vi "demo3.vi"() -> ()   [LabVIEW 2026]
uses:
  My Singleton Module.lvlib
panel:
  out "Gauge":dbl(knob) scale=0.0..10.0
  out "Status":string
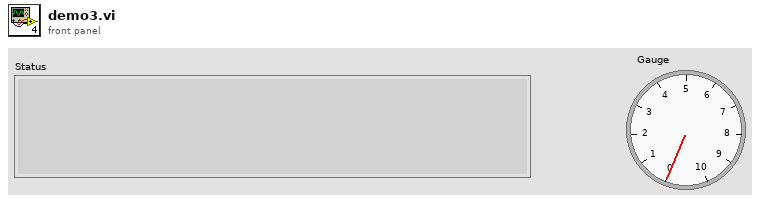
[diagram p1: front panel]
types:
  T1 = typedef "My Singleton Module.lvlib/Broadcast Events--cluster.ctl" = cluster{"Module Did Init":refnum<user-event>, "Status Updated":refnum<user-event>, "Error Reported":refnum<user-event>, "Did Something":refnum<user-event>, "Module Did Stop":refnum<user-event>, "Update Module Execution Status":refnum<user-event>, "Nuevo resultado de la Suma Actualizado":refnum<user-event>}
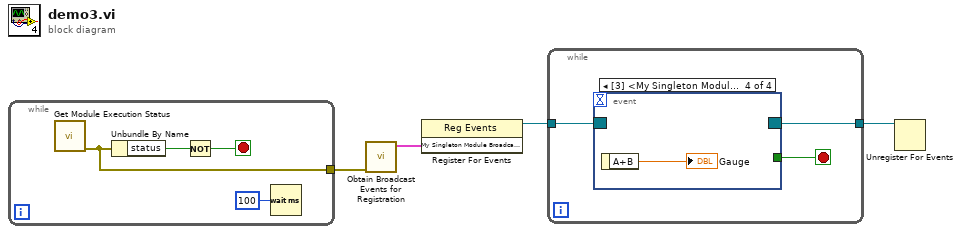
[diagram p0: block diagram]
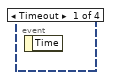
[diagram p2: hidden frame]
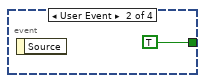
[diagram p3: hidden frame]
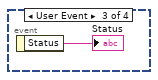
[diagram p4: hidden frame]
diagram:
  n1 = while {
    tunnel: [w5] -> w1
    stop <- w6 stop-if-true
    n2 = call "Get Module Execution Status.vi"() -> ("error out"=w5:errorcluster)  [unwired: 11 in]
    n3 = Unbundle By Name(w5) -> ("status"=w7:bool)
    n4 = Not(x=w7) -> (.not. x?=w6:bool)
    n5 = Wait (ms)(milliseconds to wait=u32 100) -> ()  [unwired: 1 out]
  }
  n6 = call "Obtain Broadcast Events for Registration.vi"("error in"=w1) -> ("My Singleton Module Broadcast Events"=w4:T1)  [unwired: 8 in, 2 out]
  n7 = register-events(w4) -> (reference out=w3:refnum<event-registration>)  [unwired: 2 in, 1 out]
  n8 = while {
    tunnel: w3 -> [w11]
    tunnel: [w9] -> w2
    stop <- w10 stop-if-true
    n9 = event shown="[3] <My Singleton Module Broadcast Events.Nuevo resultado de la Suma Actualizado>: User Event" {
      selector: w11 -> [_ _ _ _]
      dyn-events: [_ _ _ _] -> w9
      timeout: _ -> [_ _ _ _]
      tunnel: [_ TRUE _ _] -> w10
      event Timeout {
        n10 = event-data() -> ()  [unwired: 1 in, 1 out]
      }
      event User Event {
        n11 = event-data() -> ()  [unwired: 1 in, 1 out]
      }
      event User Event {
        n12 = event-data() -> ("Status"=→"Status":string)  [unwired: 1 in]
      }
      event User Event {
        n13 = event-data() -> ("A+B"=→"Gauge":dbl)  [unwired: 1 in]
      }
    }
  }
  n14 = Unregister For Events(event registration refnum=w2) -> ()  [unwired: 1 in, 1 out]
